vi "Call.vi"(8 "error in (no error)":errorcluster, 9 "Arguments":variant, 10 "Function":string, 11 "Tool in":refnum<class "ITool.lvclass">) -> (0 "error out":errorcluster, 2 "Result":variant, 3 "Tool out":refnum<class "ITool.lvclass">)   [LabVIEW 2017, in "ITool.lvclass"]
uses:
  ITool.lvclass
  <vilib>/LVH/i3 JSON/JSON Generation/Create Value Files/Create Value - Object.vi
  <vilib>/LVH/i3 JSON/JSON Generation/Add Object Parameter Files/Add Object Parameter - String.vi
  <vilib>/LVH/i3 JSON/JSON Generation/Add Object Parameter Files/Add Object Parameter - Object.vi
  <vilib>/LVH/i3 JSON/i3-json.lvlib
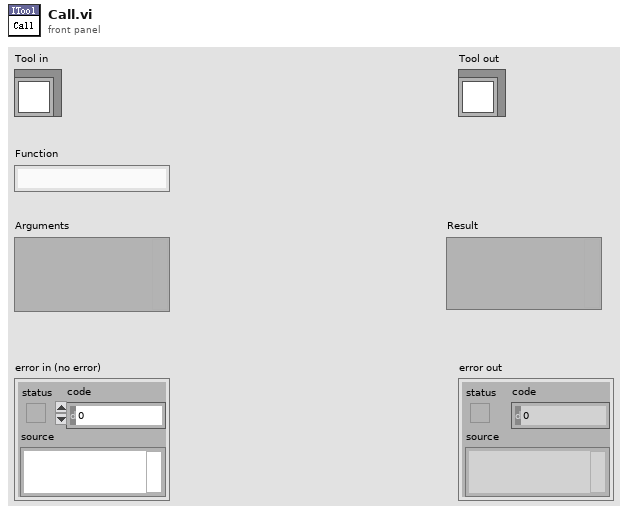
[diagram p1: front panel]
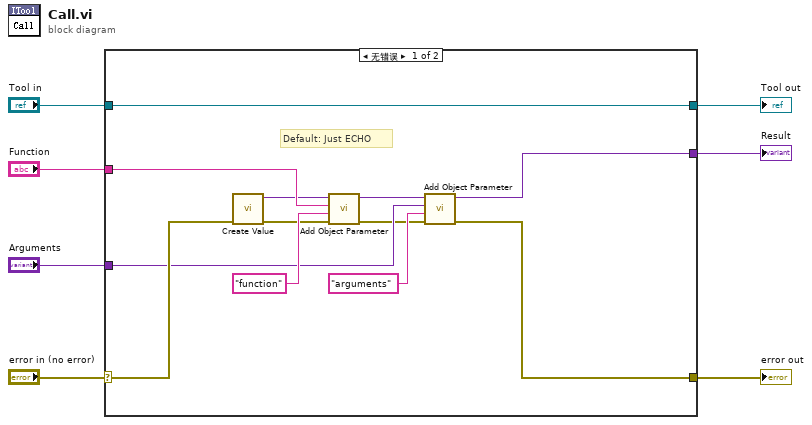
[diagram p0: block diagram]
diagram:
  n1 = case shown="无错误" "error in (no error)" {
    selector: "error in (no error)" -> [w14 w21]
    tunnel: [w9 w21] -> w4
    tunnel: [w19 w20] -> w6
    tunnel: "Tool in" -> [w19 w20]
    tunnel: "Function" -> [w17 _]
    tunnel: "Arguments" -> [w11 _]
    tunnel: [w8 _] -> w1
    frame No Error {
      # "Default: Just ECHO"
      n2 = call-poly <vilib>:"Create Value.vi"("error in (no error)"=w14) -> ("error out"=w15:errorcluster, "JSON Tree"=w16:variant)  [unwired: 9 in]
      n3 = call-poly <vilib>:"Add Object Parameter.vi"("error in (no error)"=w15, "Name"="function", "String"=w17, "JSON Tree in (JSON Object)"=w16) -> ("error out"=w10:errorcluster, "JSON Tree out (JSON Object)"=w13:variant)  [unwired: 6 in]
      n4 = call-poly <vilib>:"Add Object Parameter.vi"("error in (no error)"=w10, "Name"="arguments", "JSON Object"=w11, "JSON Tree in (JSON Object)"=w13) -> ("error out"=w9:errorcluster, "JSON Tree out (JSON Object)"=w8:variant)  [unwired: 6 in]
    }
    frame Error {
    }
  }
  "Tool out" <- w6
  "error out" <- w4
  "Result" <- w1
